vi "Write Server RPC Methods.vi"(8 "error in (no error)":errorcluster, 10 "Server RPC Methods":T1, 11 "gRPC service in":refnum<class "CanWriterCansub.lvclass">) -> (0 "error out":errorcluster, 3 "gRPC service out":refnum<class "CanWriterCansub.lvclass">)   [LabVIEW 2021, in "CanWriterCansub_server.lvlib" / "CanWriterCansub.lvclass"]
uses:
  CanWriterCansub.lvclass
  typeDefs/Server gRPC UEs.ctl
  <vilib>/gRPC/LabVIEW gRPC Library/Server API/typeDefs/gRPCId Cluster.ctl
  <vilib>/gRPC/LabVIEW gRPC Library/Shared/grpcId.ctl
  CanWriterCansub.lvclass/CanWriterCansub.ctl
  <vilib>/gRPC/LabVIEW gRPC Library/grpc-lvsupport-release.lvlib
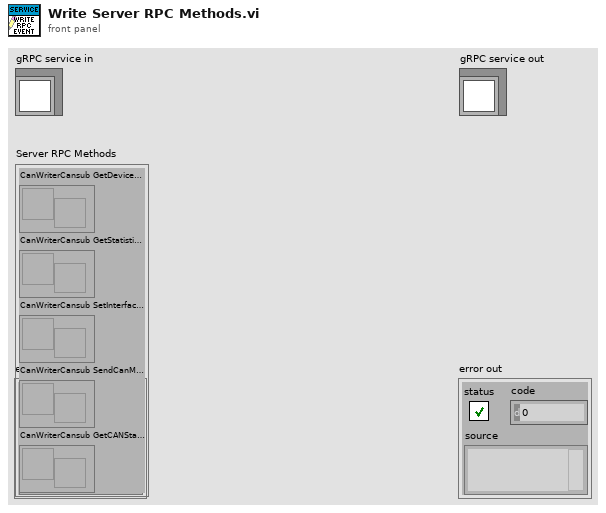
[diagram p1: front panel]
types:
  T1 = typedef "CanWriterCansub_server.lvlib/CanWriterCansub.lvclass/Server gRPC UEs.ctl" = cluster{"CanWriterCansub GetDevices gRPC UE":refnum<user-event>, "CanWriterCansub GetStatistics gRPC UE":refnum<user-event>, "CanWriterCansub SetInterfaceBlink gRPC UE":refnum<user-event>, "CanWriterCansub SendCanMessage gRPC UE":refnum<user-event>, "CanWriterCansub GetCANStatus gRPC UE":refnum<user-event>}
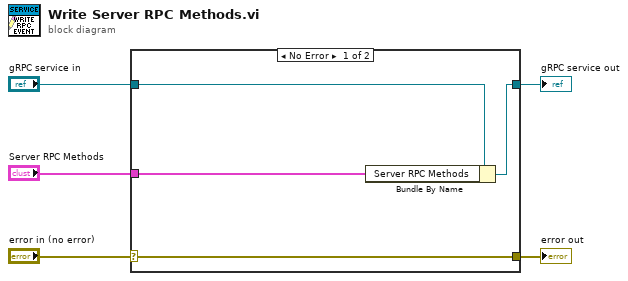
[diagram p0: block diagram]
diagram:
  n1 = case shown="No Error" "error in (no error)" {
    selector: "error in (no error)" -> [w9 w10]
    tunnel: [w9 w10] -> w4
    tunnel: [w7 w11] -> w2
    tunnel: "gRPC service in" -> [w8 w11]
    tunnel: "Server RPC Methods" -> [w6 _]
    frame No Error {
      n2 = Bundle By Name(cluster=w8, "Server RPC Methods"=w6) -> (w7:refnum<class "CanWriterCansub.lvclass">)
    }
    frame Error {
    }
  }
  "error out" <- w4
  "gRPC service out" <- w2
